vi "KYFG Camera Info.vi"(8 "error in (no error)":errorcluster, 10 "info":T1={"master_link"=0, "link_mask"=0, "@dummy control@"=0, "@dummy control@"=0, "link_speed"=40, "stream_id"=0, "deviceVersion[0]"=0, "deviceVersion[1]"=0, "deviceVersion[2]"=0, "deviceVersion[3]"=0, "deviceVersion[4]"=0, "deviceVersion[5]"=0, "deviceVersion[6]"=0, "deviceVersion[7]"=0, "deviceVersion[8]"=0, "deviceVersion[9]"=0, "deviceVersion[10]"=0, "deviceVersion[11]"=0, "deviceVersion[12]"=0, "deviceVersion[13]"=0, "deviceVersion[14]"=0, "deviceVersion[15]"=0, "deviceVersion[16]"=0, "deviceVersion[17]"=0, "deviceVersion[18]"=0, "deviceVersion[19]"=0, "deviceVersion[20]"=0, "deviceVersion[21]"=0, "deviceVersion[22]"=0, "deviceVersion[23]"=0, "deviceVersion[24]"=0, "deviceVersion[25]"=0, "deviceVersion[26]"=0, "deviceVersion[27]"=0, "deviceVersion[28]"=0, "deviceVersion[29]"=0, "deviceVersion[30]"=0, "deviceVersion[31]"=0, "deviceVersion[32]"=0, "deviceVendorName[0]"=0, "deviceVendorName[1]"=0, "deviceVendorName[2]"=0, "deviceVendorName[3]"=0, "deviceVendorName[4]"=0, "deviceVendorName[5]"=0, "deviceVendorName[6]"=0, "deviceVendorName[7]"=0, "deviceVendorName[8]"=0, "deviceVendorName[9]"=0, "deviceVendorName[10]"=0, "deviceVendorName[11]"=0, "deviceVendorName[12]"=0, "deviceVendorName[13]"=0, "deviceVendorName[14]"=0, "deviceVendorName[15]"=0, "deviceVendorName[16]"=0, "deviceVendorName[17]"=0, "deviceVendorName[18]"=0, "deviceVendorName[19]"=0, "deviceVendorName[20]"=0, "deviceVendorName[21]"=0, "deviceVendorName[22]"=0, "deviceVendorName[23]"=0, "deviceVendorName[24]"=0, "deviceVendorName[25]"=0, "deviceVendorName[26]"=0, "deviceVendorName[27]"=0, "deviceVendorName[28]"=0, "deviceVendorName[29]"=0, "deviceVendorName[30]"=0, "deviceVendorName[31]"=0, "deviceVendorName[32]"=0, "deviceManufacturerInfo[0]"=0, "deviceManufacturerInfo[1]"=0, "deviceManufacturerInfo[2]"=0, "deviceManufacturerInfo[3]"=0, "deviceManufacturerInfo[4]"=0, "deviceManufacturerInfo[5]"=0, "deviceManufacturerInfo[6]"=0, "deviceManufacturerInfo[7]"=0, "deviceManufacturerInfo[8]"=0, "deviceManufacturerInfo[9]"=0, "deviceManufacturerInfo[10]"=0, "deviceManufacturerInfo[11]"=0, "deviceManufacturerInfo[12]"=0, "deviceManufacturerInfo[13]"=0, "deviceManufacturerInfo[14]"=0, "deviceManufacturerInfo[15]"=0, "deviceManufacturerInfo[16]"=0, "deviceManufacturerInfo[17]"=0, "deviceManufacturerInfo[18]"=0, "deviceManufacturerInfo[19]"=0, "deviceManufacturerInfo[20]"=0, "deviceManufacturerInfo[21]"=0, "deviceManufacturerInfo[22]"=0, "deviceManufacturerInfo[23]"=0, "deviceManufacturerInfo[24]"=0, "deviceManufacturerInfo[25]"=0, "deviceManufacturerInfo[26]"=0, "deviceManufacturerInfo[27]"=0, "deviceManufacturerInfo[28]"=0, "deviceManufacturerInfo[29]"=0, "deviceManufacturerInfo[30]"=0, "deviceManufacturerInfo[31]"=0, "deviceManufacturerInfo[32]"=0, "deviceManufacturerInfo[33]"=0, "deviceManufacturerInfo[34]"=0, "deviceManufacturerInfo[35]"=0, "deviceManufacturerInfo[36]"=0, "deviceManufacturerInfo[37]"=0, "deviceManufacturerInfo[38]"=0, "deviceManufacturerInfo[39]"=0, "deviceManufacturerInfo[40]"=0, "deviceManufacturerInfo[41]"=0, "deviceManufacturerInfo[42]"=0, "deviceManufacturerInfo[43]"=0, "deviceManufacturerInfo[44]"=0, "deviceManufacturerInfo[45]"=0, "deviceManufacturerInfo[46]"=0, "deviceManufacturerInfo[47]"=0, "deviceManufacturerInfo[48]"=0, "deviceModelName[0]"=0, "deviceModelName[1]"=0, "deviceModelName[2]"=0, "deviceModelName[3]"=0, "deviceModelName[4]"=0, "deviceModelName[5]"=0, "deviceModelName[6]"=0, "deviceModelName[7]"=0, "deviceModelName[8]"=0, "deviceModelName[9]"=0, "deviceModelName[10]"=0, "deviceModelName[11]"=0, "deviceModelName[12]"=0, "deviceModelName[13]"=0, "deviceModelName[14]"=0, "deviceModelName[15]"=0, "deviceModelName[16]"=0, "deviceModelName[17]"=0, "deviceModelName[18]"=0, "deviceModelName[19]"=0, "deviceModelName[20]"=0, "deviceModelName[21]"=0, "deviceModelName[22]"=0, "deviceModelName[23]"=0, "deviceModelName[24]"=0, "deviceModelName[25]"=0, "deviceModelName[26]"=0, "deviceModelName[27]"=0, "deviceModelName[28]"=0, "deviceModelName[29]"=0, "deviceModelName[30]"=0, "deviceModelName[31]"=0, "deviceModelName[32]"=0, "deviceID[0]"=0, "deviceID[1]"=0, "deviceID[2]"=0, "deviceID[3]"=0, "deviceID[4]"=0, "deviceID[5]"=0, "deviceID[6]"=0, "deviceID[7]"=0, "deviceID[8]"=0, "deviceID[9]"=0, "deviceID[10]"=0, "deviceID[11]"=0, "deviceID[12]"=0, "deviceID[13]"=0, "deviceID[14]"=0, "deviceID[15]"=0, "deviceID[16]"=0, "deviceUserID[0]"=0, "deviceUserID[1]"=0, "deviceUserID[2]"=0, "deviceUserID[3]"=0, "deviceUserID[4]"=0, "deviceUserID[5]"=0, "deviceUserID[6]"=0, "deviceUserID[7]"=0, "deviceUserID[8]"=0, "deviceUserID[9]"=0, "deviceUserID[10]"=0, "deviceUserID[11]"=0, "deviceUserID[12]"=0, "deviceUserID[13]"=0, "deviceUserID[14]"=0, "deviceUserID[15]"=0, "deviceUserID[16]"=0} {"link_speed" items=["LINK_SPEED_CXP1"=40, "LINK_SPEED_CXP2"=48, "LINK_SPEED_CXP3"=56, "LINK_SPEED_CXP5"=64, "LINK_SPEED_CXP6"=72, "LINK_SPEED_CXP10"=80, "LINK_SPEED_CXP12"=88]}, 11 "camHandle":u32) -> (0 "error out":errorcluster, 2 "info out":T1={"master_link"=0, "link_mask"=0, "@dummy control@"=0, "@dummy control@"=0, "link_speed"=40, "stream_id"=0, "deviceVersion[0]"=0, "deviceVersion[1]"=0, "deviceVersion[2]"=0, "deviceVersion[3]"=0, "deviceVersion[4]"=0, "deviceVersion[5]"=0, "deviceVersion[6]"=0, "deviceVersion[7]"=0, "deviceVersion[8]"=0, "deviceVersion[9]"=0, "deviceVersion[10]"=0, "deviceVersion[11]"=0, "deviceVersion[12]"=0, "deviceVersion[13]"=0, "deviceVersion[14]"=0, "deviceVersion[15]"=0, "deviceVersion[16]"=0, "deviceVersion[17]"=0, "deviceVersion[18]"=0, "deviceVersion[19]"=0, "deviceVersion[20]"=0, "deviceVersion[21]"=0, "deviceVersion[22]"=0, "deviceVersion[23]"=0, "deviceVersion[24]"=0, "deviceVersion[25]"=0, "deviceVersion[26]"=0, "deviceVersion[27]"=0, "deviceVersion[28]"=0, "deviceVersion[29]"=0, "deviceVersion[30]"=0, "deviceVersion[31]"=0, "deviceVersion[32]"=0, "deviceVendorName[0]"=0, "deviceVendorName[1]"=0, "deviceVendorName[2]"=0, "deviceVendorName[3]"=0, "deviceVendorName[4]"=0, "deviceVendorName[5]"=0, "deviceVendorName[6]"=0, "deviceVendorName[7]"=0, "deviceVendorName[8]"=0, "deviceVendorName[9]"=0, "deviceVendorName[10]"=0, "deviceVendorName[11]"=0, "deviceVendorName[12]"=0, "deviceVendorName[13]"=0, "deviceVendorName[14]"=0, "deviceVendorName[15]"=0, "deviceVendorName[16]"=0, "deviceVendorName[17]"=0, "deviceVendorName[18]"=0, "deviceVendorName[19]"=0, "deviceVendorName[20]"=0, "deviceVendorName[21]"=0, "deviceVendorName[22]"=0, "deviceVendorName[23]"=0, "deviceVendorName[24]"=0, "deviceVendorName[25]"=0, "deviceVendorName[26]"=0, "deviceVendorName[27]"=0, "deviceVendorName[28]"=0, "deviceVendorName[29]"=0, "deviceVendorName[30]"=0, "deviceVendorName[31]"=0, "deviceVendorName[32]"=0, "deviceManufacturerInfo[0]"=0, "deviceManufacturerInfo[1]"=0, "deviceManufacturerInfo[2]"=0, "deviceManufacturerInfo[3]"=0, "deviceManufacturerInfo[4]"=0, "deviceManufacturerInfo[5]"=0, "deviceManufacturerInfo[6]"=0, "deviceManufacturerInfo[7]"=0, "deviceManufacturerInfo[8]"=0, "deviceManufacturerInfo[9]"=0, "deviceManufacturerInfo[10]"=0, "deviceManufacturerInfo[11]"=0, "deviceManufacturerInfo[12]"=0, "deviceManufacturerInfo[13]"=0, "deviceManufacturerInfo[14]"=0, "deviceManufacturerInfo[15]"=0, "deviceManufacturerInfo[16]"=0, "deviceManufacturerInfo[17]"=0, "deviceManufacturerInfo[18]"=0, "deviceManufacturerInfo[19]"=0, "deviceManufacturerInfo[20]"=0, "deviceManufacturerInfo[21]"=0, "deviceManufacturerInfo[22]"=0, "deviceManufacturerInfo[23]"=0, "deviceManufacturerInfo[24]"=0, "deviceManufacturerInfo[25]"=0, "deviceManufacturerInfo[26]"=0, "deviceManufacturerInfo[27]"=0, "deviceManufacturerInfo[28]"=0, "deviceManufacturerInfo[29]"=0, "deviceManufacturerInfo[30]"=0, "deviceManufacturerInfo[31]"=0, "deviceManufacturerInfo[32]"=0, "deviceManufacturerInfo[33]"=0, "deviceManufacturerInfo[34]"=0, "deviceManufacturerInfo[35]"=0, "deviceManufacturerInfo[36]"=0, "deviceManufacturerInfo[37]"=0, "deviceManufacturerInfo[38]"=0, "deviceManufacturerInfo[39]"=0, "deviceManufacturerInfo[40]"=0, "deviceManufacturerInfo[41]"=0, "deviceManufacturerInfo[42]"=0, "deviceManufacturerInfo[43]"=0, "deviceManufacturerInfo[44]"=0, "deviceManufacturerInfo[45]"=0, "deviceManufacturerInfo[46]"=0, "deviceManufacturerInfo[47]"=0, "deviceManufacturerInfo[48]"=0, "deviceModelName[0]"=0, "deviceModelName[1]"=0, "deviceModelName[2]"=0, "deviceModelName[3]"=0, "deviceModelName[4]"=0, "deviceModelName[5]"=0, "deviceModelName[6]"=0, "deviceModelName[7]"=0, "deviceModelName[8]"=0, "deviceModelName[9]"=0, "deviceModelName[10]"=0, "deviceModelName[11]"=0, "deviceModelName[12]"=0, "deviceModelName[13]"=0, "deviceModelName[14]"=0, "deviceModelName[15]"=0, "deviceModelName[16]"=0, "deviceModelName[17]"=0, "deviceModelName[18]"=0, "deviceModelName[19]"=0, "deviceModelName[20]"=0, "deviceModelName[21]"=0, "deviceModelName[22]"=0, "deviceModelName[23]"=0, "deviceModelName[24]"=0, "deviceModelName[25]"=0, "deviceModelName[26]"=0, "deviceModelName[27]"=0, "deviceModelName[28]"=0, "deviceModelName[29]"=0, "deviceModelName[30]"=0, "deviceModelName[31]"=0, "deviceModelName[32]"=0, "deviceID[0]"=0, "deviceID[1]"=0, "deviceID[2]"=0, "deviceID[3]"=0, "deviceID[4]"=0, "deviceID[5]"=0, "deviceID[6]"=0, "deviceID[7]"=0, "deviceID[8]"=0, "deviceID[9]"=0, "deviceID[10]"=0, "deviceID[11]"=0, "deviceID[12]"=0, "deviceID[13]"=0, "deviceID[14]"=0, "deviceID[15]"=0, "deviceID[16]"=0, "deviceUserID[0]"=0, "deviceUserID[1]"=0, "deviceUserID[2]"=0, "deviceUserID[3]"=0, "deviceUserID[4]"=0, "deviceUserID[5]"=0, "deviceUserID[6]"=0, "deviceUserID[7]"=0, "deviceUserID[8]"=0, "deviceUserID[9]"=0, "deviceUserID[10]"=0, "deviceUserID[11]"=0, "deviceUserID[12]"=0, "deviceUserID[13]"=0, "deviceUserID[14]"=0, "deviceUserID[15]"=0, "deviceUserID[16]"=0} {"link_speed" items=["LINK_SPEED_CXP1"=40, "LINK_SPEED_CXP2"=48, "LINK_SPEED_CXP3"=56, "LINK_SPEED_CXP5"=64, "LINK_SPEED_CXP6"=72, "LINK_SPEED_CXP10"=80, "LINK_SPEED_CXP12"=88]}, 3 "function return":u32(ring))   [LabVIEW 2023, in "KYFGLib_lv.lvlib"]
doc: "KYFG_API FGSTATUS KYFG_CameraInfo(CAMHANDLE camHandle, KYFGCAMERA_INFO *info);"
uses:
  KYFGLib_lv.lvlib
  KYFGLib.dll
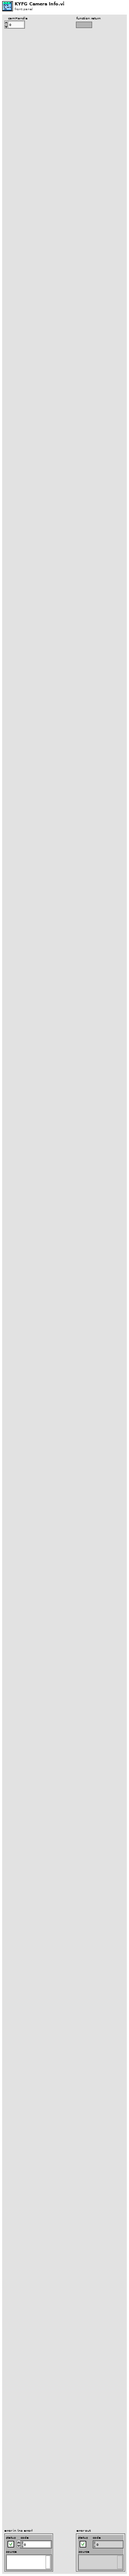
[diagram p1: front panel]
types:
  T1 = cluster{"master_link":u8, "link_mask":u8, "@dummy control@":i8, "@dummy control@":i8, "link_speed":u32, "stream_id":u32, "deviceVersion[0]":i8, "deviceVersion[1]":i8, "deviceVersion[2]":i8, "deviceVersion[3]":i8, "deviceVersion[4]":i8, "deviceVersion[5]":i8, "deviceVersion[6]":i8, "deviceVersion[7]":i8, "deviceVersion[8]":i8, "deviceVersion[9]":i8, "deviceVersion[10]":i8, "deviceVersion[11]":i8, "deviceVersion[12]":i8, "deviceVersion[13]":i8, "deviceVersion[14]":i8, "deviceVersion[15]":i8, "deviceVersion[16]":i8, "deviceVersion[17]":i8, "deviceVersion[18]":i8, "deviceVersion[19]":i8, "deviceVersion[20]":i8, "deviceVersion[21]":i8, "deviceVersion[22]":i8, "deviceVersion[23]":i8, "deviceVersion[24]":i8, "deviceVersion[25]":i8, "deviceVersion[26]":i8, "deviceVersion[27]":i8, "deviceVersion[28]":i8, "deviceVersion[29]":i8, "deviceVersion[30]":i8, "deviceVersion[31]":i8, "deviceVersion[32]":i8, "deviceVendorName[0]":i8, "deviceVendorName[1]":i8, "deviceVendorName[2]":i8, "deviceVendorName[3]":i8, "deviceVendorName[4]":i8, "deviceVendorName[5]":i8, "deviceVendorName[6]":i8, "deviceVendorName[7]":i8, "deviceVendorName[8]":i8, "deviceVendorName[9]":i8, "deviceVendorName[10]":i8, "deviceVendorName[11]":i8, "deviceVendorName[12]":i8, "deviceVendorName[13]":i8, "deviceVendorName[14]":i8, "deviceVendorName[15]":i8, "deviceVendorName[16]":i8, "deviceVendorName[17]":i8, "deviceVendorName[18]":i8, "deviceVendorName[19]":i8, "deviceVendorName[20]":i8, "deviceVendorName[21]":i8, "deviceVendorName[22]":i8, "deviceVendorName[23]":i8, "deviceVendorName[24]":i8, "deviceVendorName[25]":i8, "deviceVendorName[26]":i8, "deviceVendorName[27]":i8, "deviceVendorName[28]":i8, "deviceVendorName[29]":i8, "deviceVendorName[30]":i8, "deviceVendorName[31]":i8, "deviceVendorName[32]":i8, "deviceManufacturerInfo[0]":i8, "deviceManufacturerInfo[1]":i8, "deviceManufacturerInfo[2]":i8, "deviceManufacturerInfo[3]":i8, "deviceManufacturerInfo[4]":i8, "deviceManufacturerInfo[5]":i8, "deviceManufacturerInfo[6]":i8, "deviceManufacturerInfo[7]":i8, "deviceManufacturerInfo[8]":i8, "deviceManufacturerInfo[9]":i8, "deviceManufacturerInfo[10]":i8, "deviceManufacturerInfo[11]":i8, "deviceManufacturerInfo[12]":i8, "deviceManufacturerInfo[13]":i8, "deviceManufacturerInfo[14]":i8, "deviceManufacturerInfo[15]":i8, "deviceManufacturerInfo[16]":i8, "deviceManufacturerInfo[17]":i8, "deviceManufacturerInfo[18]":i8, "deviceManufacturerInfo[19]":i8, "deviceManufacturerInfo[20]":i8, "deviceManufacturerInfo[21]":i8, "deviceManufacturerInfo[22]":i8, "deviceManufacturerInfo[23]":i8, "deviceManufacturerInfo[24]":i8, "deviceManufacturerInfo[25]":i8, "deviceManufacturerInfo[26]":i8, "deviceManufacturerInfo[27]":i8, "deviceManufacturerInfo[28]":i8, "deviceManufacturerInfo[29]":i8, "deviceManufacturerInfo[30]":i8, "deviceManufacturerInfo[31]":i8, "deviceManufacturerInfo[32]":i8, "deviceManufacturerInfo[33]":i8, "deviceManufacturerInfo[34]":i8, "deviceManufacturerInfo[35]":i8, "deviceManufacturerInfo[36]":i8, "deviceManufacturerInfo[37]":i8, "deviceManufacturerInfo[38]":i8, "deviceManufacturerInfo[39]":i8, "deviceManufacturerInfo[40]":i8, "deviceManufacturerInfo[41]":i8, "deviceManufacturerInfo[42]":i8, "deviceManufacturerInfo[43]":i8, "deviceManufacturerInfo[44]":i8, "deviceManufacturerInfo[45]":i8, "deviceManufacturerInfo[46]":i8, "deviceManufacturerInfo[47]":i8, "deviceManufacturerInfo[48]":i8, "deviceModelName[0]":i8, "deviceModelName[1]":i8, "deviceModelName[2]":i8, "deviceModelName[3]":i8, "deviceModelName[4]":i8, "deviceModelName[5]":i8, "deviceModelName[6]":i8, "deviceModelName[7]":i8, "deviceModelName[8]":i8, "deviceModelName[9]":i8, "deviceModelName[10]":i8, "deviceModelName[11]":i8, "deviceModelName[12]":i8, "deviceModelName[13]":i8, "deviceModelName[14]":i8, "deviceModelName[15]":i8, "deviceModelName[16]":i8, "deviceModelName[17]":i8, "deviceModelName[18]":i8, "deviceModelName[19]":i8, "deviceModelName[20]":i8, "deviceModelName[21]":i8, "deviceModelName[22]":i8, "deviceModelName[23]":i8, "deviceModelName[24]":i8, "deviceModelName[25]":i8, "deviceModelName[26]":i8, "deviceModelName[27]":i8, "deviceModelName[28]":i8, "deviceModelName[29]":i8, "deviceModelName[30]":i8, "deviceModelName[31]":i8, "deviceModelName[32]":i8, "deviceID[0]":i8, "deviceID[1]":i8, "deviceID[2]":i8, "deviceID[3]":i8, "deviceID[4]":i8, "deviceID[5]":i8, "deviceID[6]":i8, "deviceID[7]":i8, "deviceID[8]":i8, "deviceID[9]":i8, "deviceID[10]":i8, "deviceID[11]":i8, "deviceID[12]":i8, "deviceID[13]":i8, "deviceID[14]":i8, "deviceID[15]":i8, "deviceID[16]":i8, "deviceUserID[0]":i8, "deviceUserID[1]":i8, "deviceUserID[2]":i8, "deviceUserID[3]":i8, "deviceUserID[4]":i8, "deviceUserID[5]":i8, "deviceUserID[6]":i8, "deviceUserID[7]":i8, "deviceUserID[8]":i8, "deviceUserID[9]":i8, "deviceUserID[10]":i8, "deviceUserID[11]":i8, "deviceUserID[12]":i8, "deviceUserID[13]":i8, "deviceUserID[14]":i8, "deviceUserID[15]":i8, "deviceUserID[16]":i8}
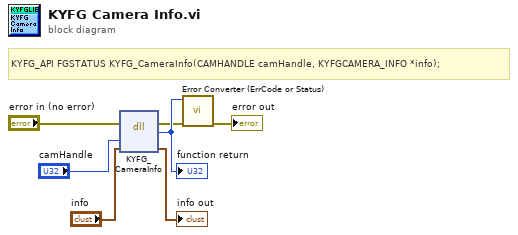
[diagram p0: block diagram]
diagram:
  # "KYFG_API FGSTATUS KYFG_CameraInfo(CAMHANDLE camHandle, KYFGCAMERA_INFO *info);"
  n1 = dll-call lib="KYFGLib.dll" fn="KYFG_CameraInfo"(error in="error in (no error)", "camHandle"="camHandle", "info"="info") -> (error out=w2:errorcluster, "return type"=w7:u32, "info"=→"info out":T1)  [unwired: 3 in, 1 out]
  "function return" <- w7
  n2 = call "Error Converter (ErrCode or Status).vi"("error in (no error)"=w2, "error code"=w7) -> ("error out"=→"error out":errorcluster)  [unwired: 9 in]
